vi "Registry_Init.vi"(8 "error in (no error)":errorcluster={"status"=FALSE, "code"=0, "source"="\"\""}, 10 "clock policy":string, 11 "RigDefinition":string) -> (0 "error out":errorcluster={"status"=FALSE, "code"=0, "source"="\"\""}, 2 "status ok":bool, 3 "Registry context":string)   [LabVIEW 2026]
doc: "INTENT: Create typed parameter definitions. LOGIC: Allocate parameter table, type/unit/source/freshness and quality defaults."
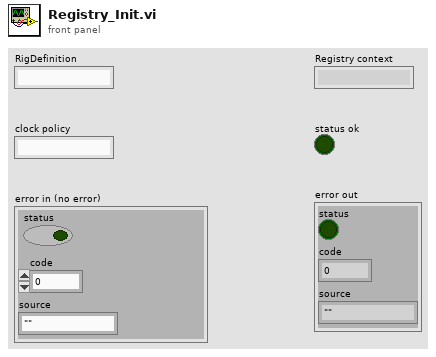
[diagram p1: front panel]
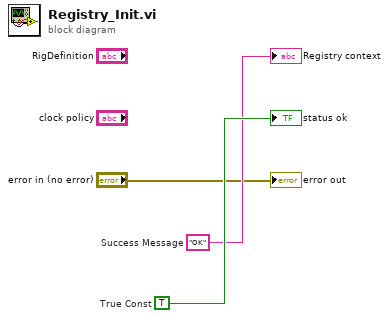
[diagram p0: block diagram]
diagram:
  w3 = TRUE  # True Const
  w2 = "OK"  # Success Message
  "Registry context" <- w2
  "status ok" <- w3
  "error out" <- "error in (no error)"
